vi "UI_Draw_Board.vi"(0 "Board State":T3={"Grid"=array15x15[225 elements], "Move History"=[], "Last Move"={"Row"=-1, "Col"=-1, "Stone"=enum."Empty"}}, 5 "Hover":T2={"Row"=-1, "Col"=-1, "Stone"=enum."Empty"}, 7 "Win Line":T1(array[cluster]), 11 "error in":errorcluster) -> (4 "Picture":picture, 15 "error out":errorcluster)   [LabVIEW 2026]
doc: "Board State를 2D Picture로 그린다: 나무 배경, 격자선 15x15, 화점 9개, 흑/백 돌(히스토리 순회), 마지막 착수 빨간 점, 호버 미리보기(회색 테두리), 승리 5목 라인(빨간 굵은 선)."
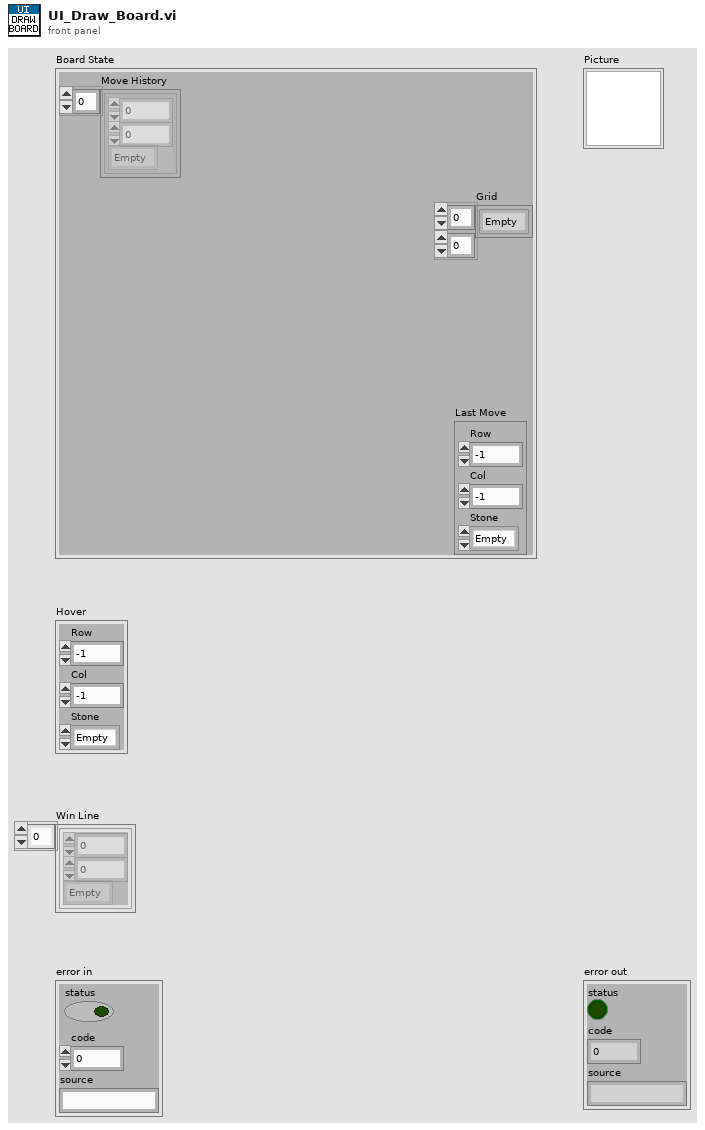
[diagram p1: front panel]
types:
  T1 = cluster{"Row":i32, "Col":i32, "Stone":enum8{"Empty", "Black", "White"}}[]
  T2 = cluster{"Row":i32, "Col":i32, "Stone":enum8{"Empty", "Black", "White"}}
  T3 = cluster{"Grid":enum8{"Empty", "Black", "White"}[][], "Move History":cluster{"Row":i32, "Col":i32, "Stone":enum8{"Empty", "Black", "White"}}[], "Last Move":cluster{"Row":i32, "Col":i32, "Stone":enum8{"Empty", "Black", "White"}}}
  T4 = cluster{"left":i16, "top":i16, "right":i16, "bottom":i16}
  T5 = cluster{"Width":u16, "Style":enum32{"Solid", "Dash", "Dot", "DashDot", "DashDotDot"}}
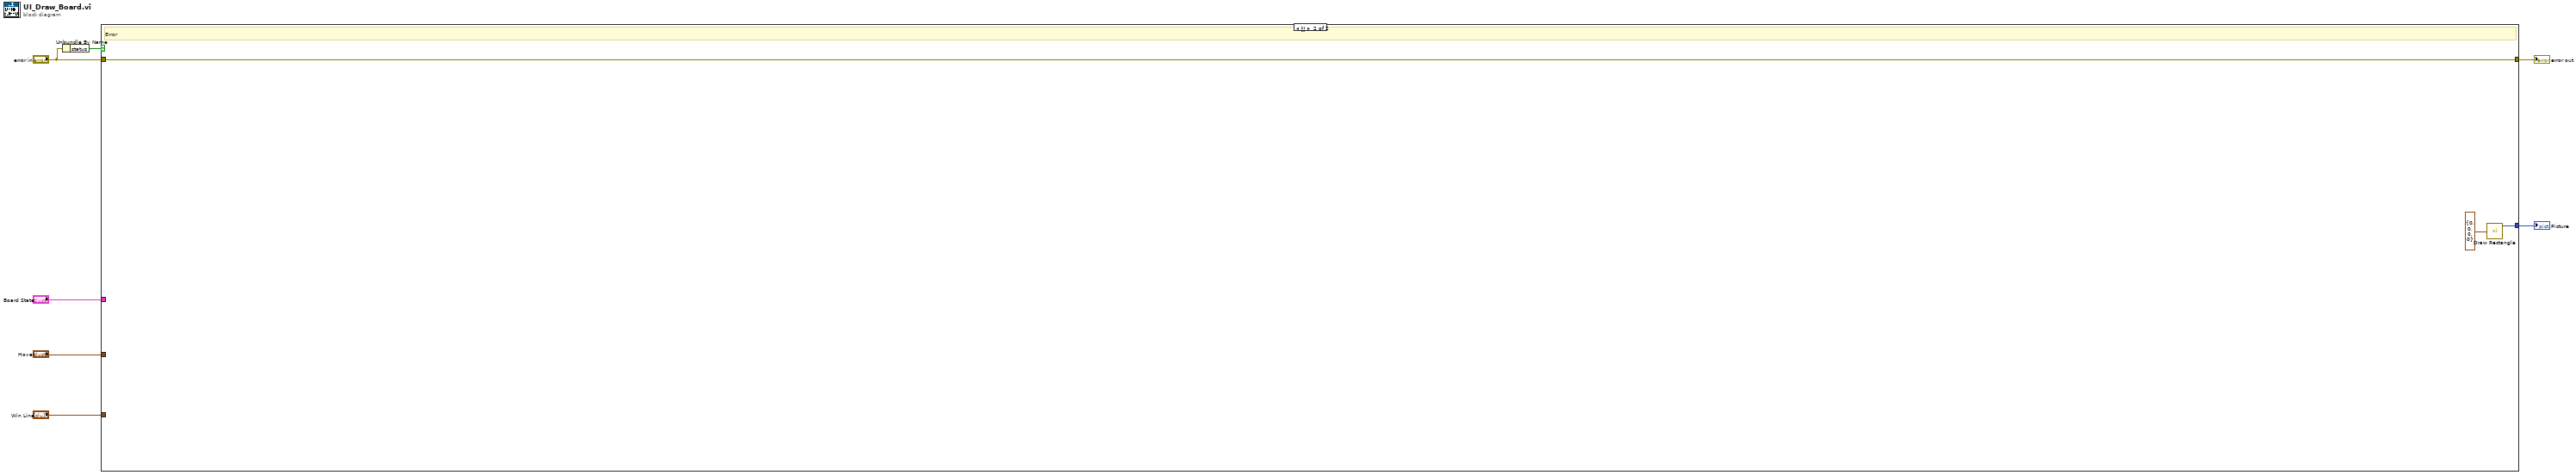
[diagram p0: block diagram]
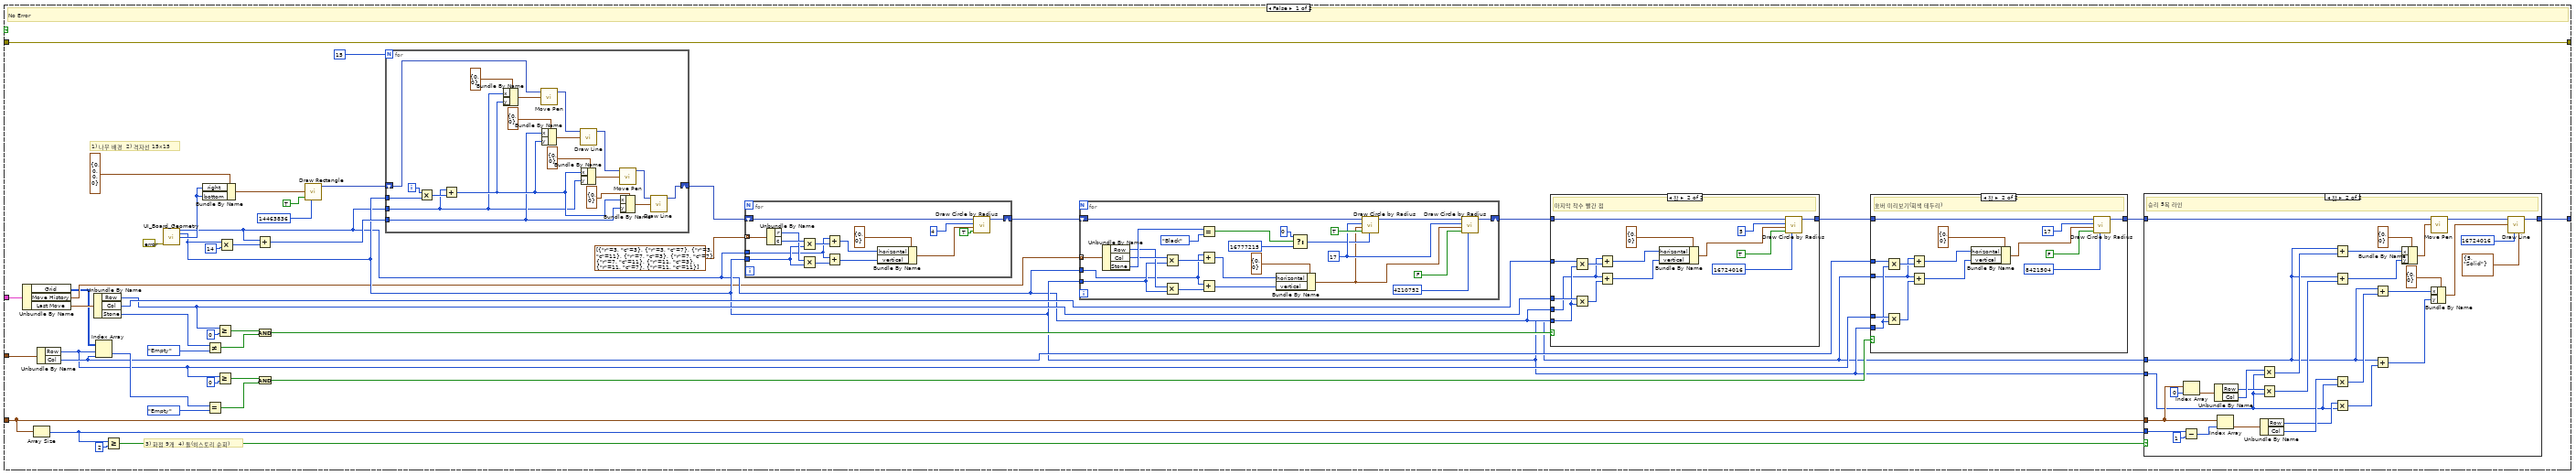
[diagram p2: hidden frame]
diagram:
  n1 = Unbundle By Name("error in") -> ("status"=w5:bool)
  n2 = case shown="참" w5 {
    tunnel: "Board State" -> [w8 _]
    tunnel: "Hover" -> [w9 _]
    tunnel: "Win Line" -> [w10 _]
    tunnel: "error in" -> [w11 w175]
    tunnel: [w11 w175] -> w7
    tunnel: [w53 w177] -> w6
    frame False {
      # "3) 화점 9개  4) 돌(히스토리 순회)"
      # "1) 나무 배경  2) 격자선 15x15"
      # "No Error"
      n3 = Unbundle By Name(w8) -> ("Grid"=w12:enum8{"Empty", "Black", "White"}[][], "Move History"=w13:T1, "Last Move"=w14:T2)
      n4 = Array Size(array=w10) -> (size(s)=w50:i32)
      n5 = Unbundle By Name(w9) -> ("Row"=w41:i32, "Col"=w42:i32)
      n6 = Unbundle By Name(w14) -> ("Row"=w32:i32, "Col"=w33:i32, "Stone"=w34:enum8{"Empty", "Black", "White"})
      n7 = Index Array(array=w12, index (row)=w41, index (col)=w42) -> (element=w43:enum8{"Empty", "Black", "White"})
      n8 = Greater Or Equal?(x=w50, y=2) -> (x >= y?=w52:bool)
      n9 = call "UI_Board_Geometry.vi"("error in"=errorcluster {"status"=FALSE, "code"=0, "source"=""}) -> ("Origin"=w16:i32, "Cell"=w17:i32, "Size"=w18:i32)  [unwired: 11 in, 1 out]
      n10 = Bundle By Name(cluster=T4 {"left"=0, "top"=0, "right"=0, "bottom"=0}, "right"=w18, "bottom"=w18) -> (w20:T4)
      n11 = Not Equal?(x=w34, y=enum8{"Empty", "Black", "White"}."Empty") -> (x != y?=w38:bool)
      n12 = Equal?(x=w43, y=enum8{"Empty", "Black", "White"}."Empty") -> (x = y?=w47:bool)
      n13 = Greater Or Equal?(x=w32, y=0) -> (x >= y?=w36:bool)
      n14 = Greater Or Equal?(x=w41, y=0) -> (x >= y?=w45:bool)
      n15 = Multiply(x=w17, y=14) -> (x*y=w25:i32)
      n16 = Add(x=w16, y=w25) -> (x+y=w26:i32)
      n17 = And(x=w36, y=w38) -> (x .and. y?=w39:bool)
      n18 = And(x=w45, y=w47) -> (x .and. y?=w48:bool)
      n19 = call <vilib>:"Draw Rectangle.vi"("rect"=w20, "fill?(F)"=TRUE, "color(black)"=u32 14463836) -> ("new picture"=w23:picture)  [unwired: 6 in]
      n20 = for {
        N: 15 -> [_]
        tunnel: w16 -> [w157]
        tunnel: w17 -> [w158]
        tunnel: w26 -> [w159]
        shift-right: [w174] -> w28
        shift-left: w23 -> [w165]
        i -> [w156]
        n21 = Multiply(x=w156, y=w158) -> (x*y=w160:i32)
        n22 = Add(x=w157, y=w160) -> (x+y=w161:i32)
        n23 = Bundle By Name(cluster=cluster{"x":i16, "y":i16} {"x"=0, "y"=0}, "x"=w157, "y"=w161) -> (w163:cluster{"x":i16, "y":i16})
        n24 = call <vilib>:"Move Pen.vi"("new position"=w163, "picture"=w165) -> ("new picture"=w164:picture)  [unwired: 3 in]
        n25 = Bundle By Name(cluster=cluster{"x":i16, "y":i16} {"x"=0, "y"=0}, "x"=w159, "y"=w161) -> (w167:cluster{"x":i16, "y":i16})
        n26 = call <vilib>:"Draw Line.vi"("picture"=w164, "end point"=w167) -> ("new picture"=w168:picture)  [unwired: 7 in]
        n27 = Bundle By Name(cluster=cluster{"x":i16, "y":i16} {"x"=0, "y"=0}, "x"=w161, "y"=w157) -> (w170:cluster{"x":i16, "y":i16})
        n28 = call <vilib>:"Move Pen.vi"("new position"=w170, "picture"=w168) -> ("new picture"=w171:picture)  [unwired: 3 in]
        n29 = Bundle By Name(cluster=cluster{"x":i16, "y":i16} {"x"=0, "y"=0}, "x"=w161, "y"=w159) -> (w173:cluster{"x":i16, "y":i16})
        n30 = call <vilib>:"Draw Line.vi"("picture"=w171, "end point"=w173) -> ("new picture"=w174:picture)  [unwired: 7 in]
      }
      n31 = for {
        tunnel: cluster{"r":i32, "c":i32}[] [{"r"=3, "c"=3}, {"r"=3, "c"=7}, {"r"=3, "c"=11}, {"r"=7, "c"=3}, {"r"=7, "c"=7}, {"r"=7, "c"=11}, {"r"=11, "c"=3}, {"r"=11, "c"=7}, {"r"=11, "c"=11}] ("Star Points") -> [w143] mode=indexing
        tunnel: w16 -> [w141]
        tunnel: w17 -> [w142]
        shift-right: [w154] -> w30
        shift-left: w28 -> [w155]
        n32 = Unbundle By Name(w143) -> ("r"=w144:i32, "c"=w145:i32)
        n33 = Multiply(x=w145, y=w142) -> (x*y=w146:i32)
        n34 = Multiply(x=w144, y=w142) -> (x*y=w148:i32)
        n35 = Add(x=w141, y=w146) -> (x+y=w147:i32)
        n36 = Add(x=w141, y=w148) -> (x+y=w149:i32)
        n37 = Bundle By Name(cluster=cluster{"horizontal":i16, "vertical":i16} {"horizontal"=0, "vertical"=0}, "horizontal"=w147, "vertical"=w149) -> (w151:cluster{"horizontal":i16, "vertical":i16})
        n38 = call <vilib>:"Draw Circle by Radius.vi"("fill?(F)"=TRUE, "pixel center"=w151, "radius"=i16 4, "picture"=w155) -> ("new picture"=w154:picture)  [unwired: 7 in]
      }
      n39 = for {
        tunnel: w16 -> [w117]
        tunnel: w17 -> [w118]
        tunnel: w13 -> [w119] mode=indexing
        shift-right: [w140] -> w31
        shift-left: w30 -> [w137]
        w134 = i16 17
        n40 = Unbundle By Name(w119) -> ("Row"=w120:i32, "Col"=w121:i32, "Stone"=w122:enum8{"Empty", "Black", "White"})
        n41 = Multiply(x=w121, y=w118) -> (x*y=w123:i32)
        n42 = Multiply(x=w120, y=w118) -> (x*y=w125:i32)
        n43 = Equal?(x=w122, y=enum8{"Empty", "Black", "White"}."Black") -> (x = y?=w130:bool)
        n44 = Add(x=w117, y=w123) -> (x+y=w124:i32)
        n45 = Add(x=w117, y=w125) -> (x+y=w126:i32)
        n46 = Bundle By Name(cluster=cluster{"horizontal":i16, "vertical":i16} {"horizontal"=0, "vertical"=0}, "horizontal"=w124, "vertical"=w126) -> (w128:cluster{"horizontal":i16, "vertical":i16})
        n47 = Select(t=u32 0, s=w130, f=u32 16777215) -> (s? t:f=w133:u32)
        n48 = call <vilib>:"Draw Circle by Radius.vi"("color(black)"=w133, "fill?(F)"=TRUE, "pixel center"=w128, "radius"=w134, "picture"=w137) -> ("new picture"=w136:picture)  [unwired: 6 in]
        n49 = call <vilib>:"Draw Circle by Radius.vi"("color(black)"=u32 4210752, "fill?(F)"=FALSE, "pixel center"=w128, "radius"=w134, "picture"=w136) -> ("new picture"=w140:picture)  [unwired: 6 in]
      }
      n50 = case shown="참" w39 {
        tunnel: w16 -> [_ w103]
        tunnel: w17 -> [_ w104]
        tunnel: w32 -> [_ w105]
        tunnel: w33 -> [_ w106]
        tunnel: w31 -> [w101 w102]
        tunnel: [w101 w116] -> w40
        frame False {
        }
        frame True {
          # "마지막 착수 빨간 점"
          n51 = Multiply(x=w106, y=w104) -> (x*y=w107:i32)
          n52 = Multiply(x=w105, y=w104) -> (x*y=w109:i32)
          n53 = Add(x=w103, y=w107) -> (x+y=w108:i32)
          n54 = Add(x=w103, y=w109) -> (x+y=w110:i32)
          n55 = Bundle By Name(cluster=cluster{"horizontal":i16, "vertical":i16} {"horizontal"=0, "vertical"=0}, "horizontal"=w108, "vertical"=w110) -> (w112:cluster{"horizontal":i16, "vertical":i16})
          n56 = call <vilib>:"Draw Circle by Radius.vi"("color(black)"=u32 16724016, "fill?(F)"=TRUE, "pixel center"=w112, "radius"=i16 5, "picture"=w102) -> ("new picture"=w116:picture)  [unwired: 6 in]
        }
      }
      n57 = case shown="참" w48 {
        tunnel: w16 -> [_ w87]
        tunnel: w17 -> [_ w88]
        tunnel: w41 -> [_ w89]
        tunnel: w42 -> [_ w90]
        tunnel: w40 -> [w85 w86]
        tunnel: [w85 w100] -> w49
        frame False {
        }
        frame True {
          # "호버 미리보기(회색 테두리)"
          n58 = Multiply(x=w90, y=w88) -> (x*y=w91:i32)
          n59 = Multiply(x=w89, y=w88) -> (x*y=w93:i32)
          n60 = Add(x=w87, y=w91) -> (x+y=w92:i32)
          n61 = Add(x=w87, y=w93) -> (x+y=w94:i32)
          n62 = Bundle By Name(cluster=cluster{"horizontal":i16, "vertical":i16} {"horizontal"=0, "vertical"=0}, "horizontal"=w92, "vertical"=w94) -> (w96:cluster{"horizontal":i16, "vertical":i16})
          n63 = call <vilib>:"Draw Circle by Radius.vi"("color(black)"=u32 8421504, "fill?(F)"=FALSE, "pixel center"=w96, "radius"=i16 17, "picture"=w86) -> ("new picture"=w100:picture)  [unwired: 6 in]
        }
      }
      n64 = case shown="참" w52 {
        tunnel: w16 -> [_ w56]
        tunnel: w17 -> [_ w57]
        tunnel: w10 -> [_ w58]
        tunnel: w50 -> [_ w59]
        tunnel: w49 -> [w54 w55]
        tunnel: [w54 w84] -> w53
        frame False {
        }
        frame True {
          # "승리 5목 라인"
          n65 = Subtract(x=w59, y=1) -> (x-y=w63:i32)
          n66 = Index Array(array=w58, index=0) -> (element=w61:T2)
          n67 = Unbundle By Name(w61) -> ("Row"=w65:i32, "Col"=w66:i32)
          n68 = Index Array(array=w58, index=w63) -> (element=w64:T2)
          n69 = Unbundle By Name(w64) -> ("Row"=w67:i32, "Col"=w68:i32)
          n70 = Multiply(x=w66, y=w57) -> (x*y=w69:i32)
          n71 = Multiply(x=w65, y=w57) -> (x*y=w71:i32)
          n72 = Add(x=w56, y=w69) -> (x+y=w70:i32)
          n73 = Add(x=w56, y=w71) -> (x+y=w72:i32)
          n74 = Multiply(x=w68, y=w57) -> (x*y=w73:i32)
          n75 = Multiply(x=w67, y=w57) -> (x*y=w75:i32)
          n76 = Add(x=w56, y=w73) -> (x+y=w74:i32)
          n77 = Add(x=w56, y=w75) -> (x+y=w76:i32)
          n78 = Bundle By Name(cluster=cluster{"x":i16, "y":i16} {"x"=0, "y"=0}, "x"=w70, "y"=w72) -> (w78:cluster{"x":i16, "y":i16})
          n79 = call <vilib>:"Move Pen.vi"("new position"=w78, "picture"=w55) -> ("new picture"=w79:picture)  [unwired: 3 in]
          n80 = Bundle By Name(cluster=cluster{"x":i16, "y":i16} {"x"=0, "y"=0}, "x"=w74, "y"=w76) -> (w81:cluster{"x":i16, "y":i16})
          n81 = call <vilib>:"Draw Line.vi"("picture"=w79, "end point"=w81, "color(black)"=u32 16724016, "pen"=T5 {"Width"=5, "Style"=enum."Solid"}) -> ("new picture"=w84:picture)  [unwired: 5 in]
        }
      }
    }
    frame True {
      # "Error"
      n82 = call <vilib>:"Draw Rectangle.vi"("rect"=T4 {"left"=0, "top"=0, "right"=0, "bottom"=0}) -> ("new picture"=w177:picture)  [unwired: 8 in]
    }
  }
  "Picture" <- w6
  "error out" <- w7
